vi "Day 16-Hex to Bits Map.vi"() -> (3 "Map":map{string, string}(c390))   [LabVIEW 2021]
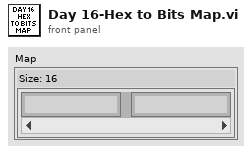
[diagram p1: front panel]
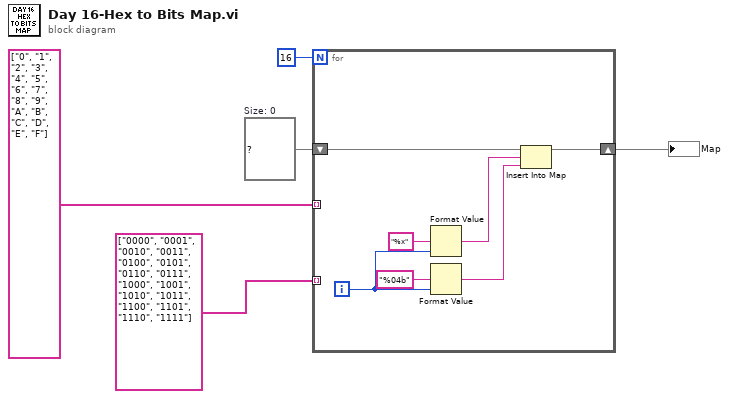
[diagram p0: block diagram]
diagram:
  w4 = map{string, string} {}  # Size: 0
  n1 = for {
    N: 16 -> [_]
    tunnel: string[] ["0", "1", "2", "3", "4", "5", "6", "7", "8", "9", "A", "B", "C", "D", "E", "F"] -> [_] mode=indexing
    tunnel: string[] ["0000", "0001", "0010", "0011", "0100", "0101", "0110", "0111", "1000", "1001", "1010", "1011", "1100", "1101", "1110", "1111"] -> [_] mode=indexing
    shift-right: [w12] -> w5
    shift-left: w4 -> [w11]
    i -> [w7]
    n2 = Format Value(format string="%x", value (0)=w7) -> (output string=w6:string)  [unwired: 1 in]
    n3 = Format Value(format string="%04b", value (0)=w7) -> (output string=w9:string)  [unwired: 1 in]
    n4 = Insert Into Map(map in=w11, key=w6, value=w9) -> (map out=w12:map{string, string})  [unwired: 2 out]
  }
  "Map" <- w5
